vi "lvmcp_gen_script_diag.vi"() -> ()   [LabVIEW 2026]
panel:
  in  "diagram":refnum<vi>
  in  "Data Strings":string[](array[string])
  in  "Type Strings":string[](array[string])
  in  "Obj Refs In[]":refnum<vi>[](array[refnum])
  out "error out":errorcluster
  out "Obj Refs Out[]":refnum<vi>[](array[refnum])
  in  "XML Script Commands":string
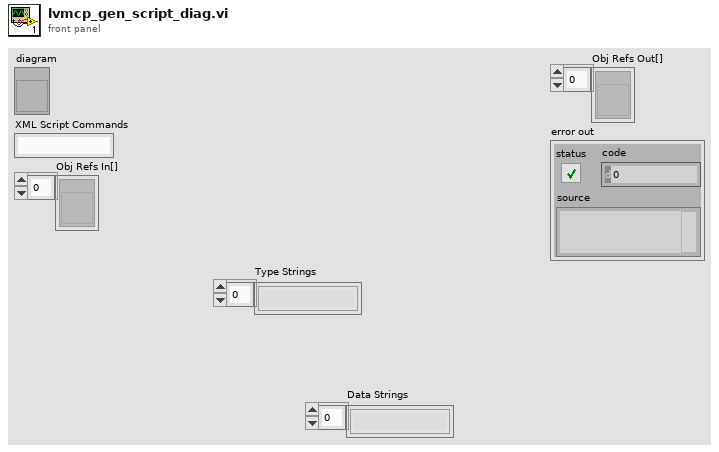
[diagram p1: front panel]
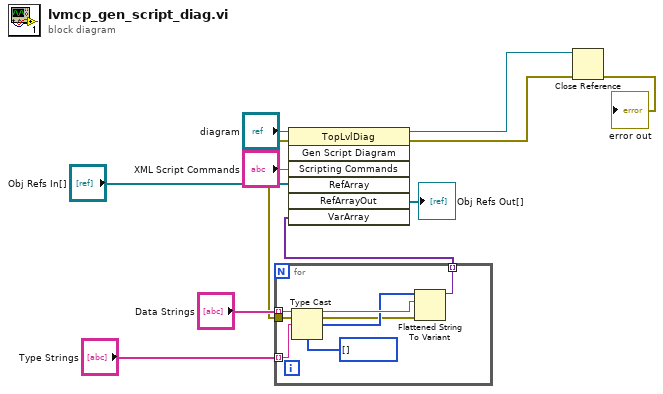
[diagram p0: block diagram]
diagram:
  n1 = for {
    tunnel: "Type Strings" -> [w16] mode=indexing
    tunnel: "Data Strings" -> [w15] mode=indexing
    tunnel: [w13] -> w5 mode=indexing
    tunnel: [w12] -> w1
    n2 = Type Cast(type=i16[] [] ("type string"), x=w16) -> (*(type *) &x=w14:i16[])
    n3 = Flattened String To Variant(6:w15, 7:w14) -> (0:w12:errorcluster, 3:w13:variant)  [unwired: 1 in]
  }
  n4 = invoke class="TopLvlDiag" method="Gen Script Diagram"(reference="diagram", error in=w1, "Scripting Commands"="XML Script Commands", "RefArray"="Obj Refs In[]", "VarArray"=w5) -> (reference out=w4:refnum<vi>, error out=w3:errorcluster, "RefArrayOut"=→"Obj Refs Out[]":refnum<vi>[])  [unwired: 2 in, 4 out]
  n5 = Close Reference(reference=w4, error in (no error)=w3) -> (error out=→"error out":errorcluster)
